vi "SID_adsr.vi"(0 "status in":T3(ring), 1 "Reg":T2, 5 "acc in":T1) -> (4 "status out":T3(ring), 6 "acc out":T1)   [LabVIEW 2018]
uses:
  SID_voice_reg.ctl
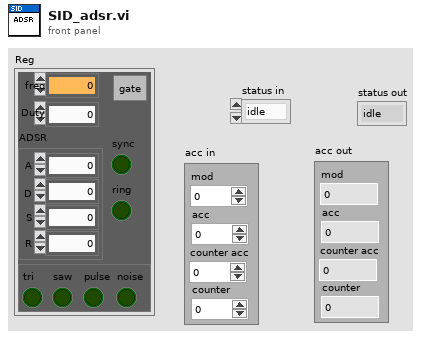
[diagram p1: front panel]
types:
  T1 = cluster{"mod":dbl, "acc":dbl, "counter acc":dbl, "counter":i32}
  T2 = typedef "SID_voice_reg.ctl" = cluster{"freq":dbl, "gate":bool, "ADSR":cluster{"A":dbl, "D":dbl, "S":dbl, "R":dbl}, "Duty":dbl, "osc enab":cluster{"tri":bool, "saw":bool, "pulse":bool, "noise":bool}, "sync":bool, "ring":bool}
  T3 = enum16{"idle", "pre-attack", "attack", "pre-decay", "decay", "sustain", "pre-release", "release"}
  T4 = cluster{"mod in":dbl, "acc in":dbl, "counter acc in":dbl, "counter in":i32}
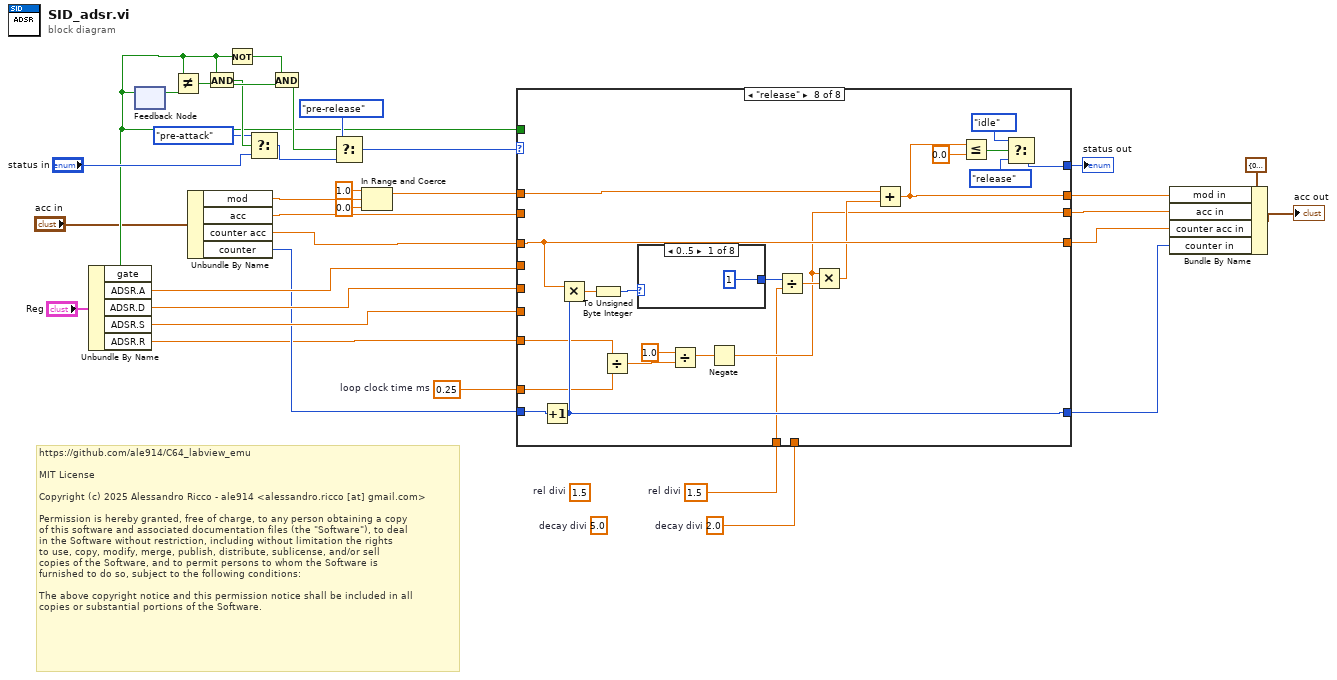
[diagram p0: block diagram]
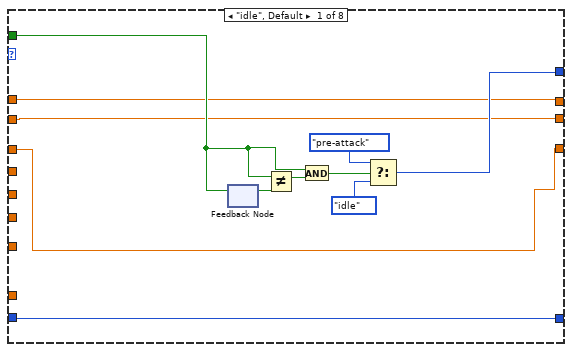
[diagram p2: hidden frame]
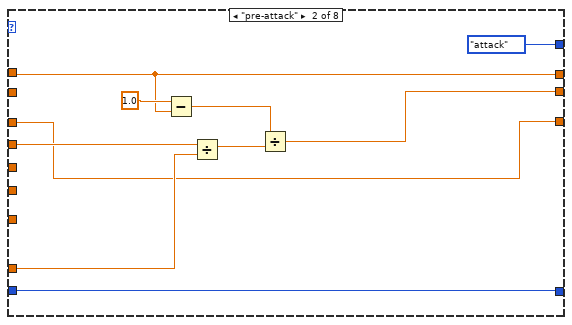
[diagram p3: hidden frame]
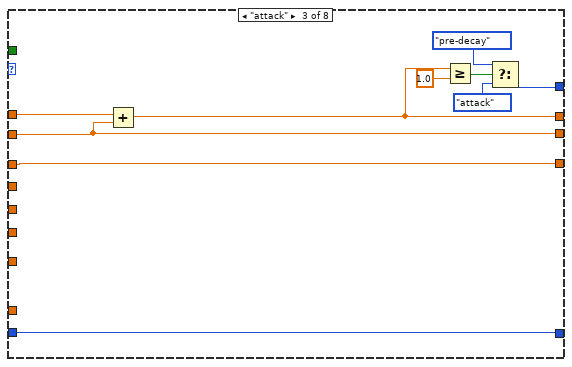
[diagram p4: hidden frame]
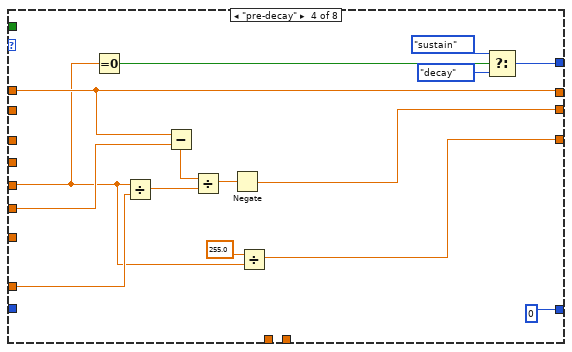
[diagram p5: hidden frame]
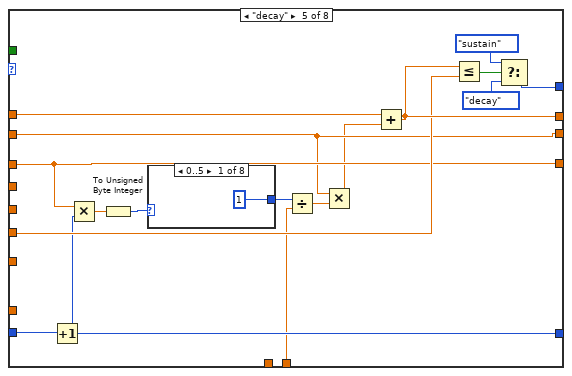
[diagram p6: hidden frame]
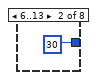
[diagram p7: hidden frame]
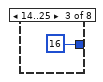
[diagram p8: hidden frame]
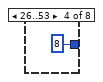
[diagram p9: hidden frame]
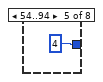
[diagram p10: hidden frame]
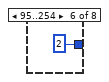
[diagram p11: hidden frame]
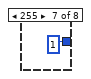
[diagram p12: hidden frame]
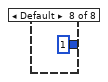
[diagram p13: hidden frame]
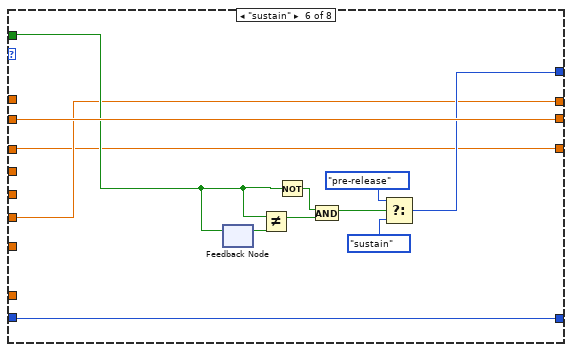
[diagram p14: hidden frame]
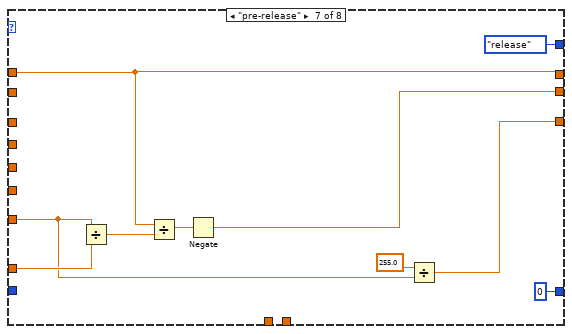
[diagram p15: hidden frame]
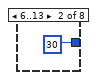
[diagram p16: hidden frame]
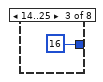
[diagram p17: hidden frame]
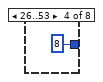
[diagram p18: hidden frame]
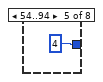
[diagram p19: hidden frame]
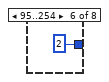
[diagram p20: hidden frame]
diagram:
  (unwired) 5.0  # decay divi
  (unwired) 1.5  # rel divi
  w1 = 2.0  # decay divi
  w2 = 1.5  # rel divi
  w22 = 0.25  # loop clock time ms
  # "https://github.com/ale914/C64_labview_emu\n\nMIT License\n\nCopyright (c) 2025 Alessandro Ricco - ale914 <alessandro.ricco [at] gmail.com>\n\nPermission is hereby granted, free of charge, to any person obtaining a copy\nof this software and associated documentation files (the \"Software\"), to deal\nin the Software without restriction, including without limitation the rights\nto use, copy, modify, merge, publish, distribute, sublicense, and/or sell\ncopies of the Software, and to permit persons to whom the Software is\nfurnished to do so, subject to the following conditions:\n\nThe above copyright notice and this permission notice shall be included in all\ncopies or substantial portions of the Software."
  n1 = Unbundle By Name("Reg") -> ("gate"=w17:bool, "ADSR.A"=w20:dbl, "ADSR.D"=w19:dbl, "ADSR.S"=w18:dbl, "ADSR.R"=w4:dbl)
  n2 = feedback #1() -> (w33:bool)  [unwired: 1 in]
  n3 = feedback-in #1(w17) -> ()
  n4 = Not Equal?(x=w17, y=w33) -> (x != y?=w32:bool)
  n5 = Unbundle By Name("acc in") -> ("mod"=w14:dbl, "acc"=w13:dbl, "counter acc"=w12:dbl, "counter"=w11:i32)
  n6 = And(x=w17, y=w32) -> (x .and. y?=w30:bool)
  n7 = Not(x=w17) -> (.not. x?=w31:bool)
  n8 = Select(t=T3."pre-attack", s=w30, f="status in") -> (s? t:f=w27:T3)
  n9 = And(x=w31, y=w32) -> (x .and. y?=w23:bool)
  n10 = Select(t=T3."pre-release", s=w23, f=w27) -> (s? t:f=w16:T3)
  n11 = In Range and Coerce(upper limit=1.0, x=w14, lower limit=0.0) -> (coerced(x)=w24:dbl)  [unwired: 1 out]
  n12 = case shown="\"release\"" w16 {
    tunnel: [w37 w55 w64 w79 w83 w117 w124 w129] -> w9
    tunnel: w13 -> [w37 _ w64 _ w83 w117 _ _]
    tunnel: w24 -> [w38 w49 w65 w73 w97 _ w118 w145]
    tunnel: [w38 w49 w63 w73 w92 w108 w118 w143] -> w10
    tunnel: [w40 T3."attack" w58 w77 w93 w109 T3."release" w144] -> w34
    tunnel: w17 -> [w39 _ _ _ _ w114 _ _]
    tunnel: w20 -> [_ w52 _ _ _ _ _ _]
    tunnel: w19 -> [_ _ _ w66 _ _ _ _]
    tunnel: w18 -> [_ _ _ w72 w91 w108 _ _]
    tunnel: w4 -> [_ _ _ _ _ _ w121 w132]
    tunnel: w22 -> [_ w51 _ w74 _ _ w123 w131]
    tunnel: [w36 w47 w57 w70 w88 w106 w120 w137] -> w8
    tunnel: w12 -> [w36 w47 w57 _ w88 w106 _ w137]
    tunnel: w11 -> [w35 w46 w56 _ w87 w107 _ w138]
    tunnel: [w35 w46 w56 0 w86 w107 0 ("counter in") w136] -> w7
    tunnel: w2 -> [_ _ _ _ _ _ _ w128]
    tunnel: w1 -> [_ _ _ _ w81 _ _ _]
    frame "idle", Default {
      n13 = feedback #2() -> (w45:bool)  [unwired: 1 in]
      n14 = feedback-in #2(w39) -> ()
      n15 = Not Equal?(x=w39, y=w45) -> (x != y?=w44:bool)
      n16 = And(x=w39, y=w44) -> (x .and. y?=w43:bool)
      n17 = Select(t=T3."pre-attack", s=w43, f=T3."idle") -> (s? t:f=w40:T3)
    }
    frame "pre-attack" {
      n18 = Subtract(x=1.0 ("y"), y=w49) -> (x-y=w48:dbl)
      n19 = Divide(x=w52, y=w51) -> (x/y=w54:dbl)
      n20 = Divide(x=w48, y=w54) -> (x/y=w55:dbl)
    }
    frame "attack" {
      n21 = Add(x=w65, y=w64) -> (x+y=w63:dbl)
      n22 = Greater Or Equal?(x=w63, y=1.0) -> (x >= y?=w59:bool)
      n23 = Select(t=T3."pre-decay", s=w59, f=T3."attack") -> (s? t:f=w58:T3)
    }
    frame "pre-decay" {
      n24 = Equal To 0?(x=w66) -> (x = 0?=w76:bool)
      n25 = Divide(x=w66, y=w74) -> (x/y=w80:dbl)
      n26 = Subtract(x=w73, y=w72) -> (x-y=w68:dbl)
      n27 = Divide(x=w68, y=w80) -> (x/y=w67:dbl)
      n28 = Negate(x=w67) -> (-x=w79:dbl)
      n29 = Divide(x=255.0 ("y"), y=w66) -> (x/y=w70:dbl)
      n30 = Select(t=T3."sustain", s=w76, f=T3."decay") -> (s? t:f=w77:T3)
    }
    frame "decay" {
      n31 = Increment(x=w87) -> (x+1=w86:i32)
      n32 = Multiply(x=w88, y=w86) -> (x*y=w85:dbl)
      n33 = To Unsigned Byte Integer(number=w85) -> (unsigned 8bit integer=w90:u8)
      n34 = case shown="0..5" w90 {
        tunnel: [u8 1 ("exp_period") u8 30 ("exp_period") u8 16 ("exp_period") u8 8 ("exp_period") u8 4 ("exp_period") u8 2 ("exp_period") u8 1 ("exp_period") u8 1 ("exp_period")] -> w89
        frame 0..5 {
          (unwired) TRUE ("hold zero")
        }
        frame 6..13 {
        }
        frame 14..25 {
        }
        frame 26..53 {
        }
        frame 54..94 {
        }
        frame 95..254 {
        }
        frame 255 {
        }
        frame Default {
        }
      }
      n35 = Divide(x=w89, y=w81) -> (x/y=w84:dbl)
      n36 = Multiply(x=w83, y=w84) -> (x*y=w82:dbl)
      n37 = Add(x=w97, y=w82) -> (x+y=w92:dbl)
      n38 = Less Or Equal?(x=w92, y=w91) -> (x <= y?=w94:bool)
      n39 = Select(t=T3."sustain", s=w94, f=T3."decay") -> (s? t:f=w93:T3)
    }
    frame "sustain" {
      n40 = feedback #3() -> (w116:bool)  [unwired: 1 in]
      n41 = feedback-in #3(w114) -> ()
      n42 = Not Equal?(x=w114, y=w116) -> (x != y?=w115:bool)
      n43 = Not(x=w114) -> (.not. x?=w113:bool)
      n44 = And(x=w113, y=w115) -> (x .and. y?=w110:bool)
      n45 = Select(t=T3."pre-release", s=w110, f=T3."sustain") -> (s? t:f=w109:T3)
    }
    frame "pre-release" {
      n46 = Divide(x=w121, y=w123) -> (x/y=w126:dbl)
      n47 = Divide(x=w118, y=w126) -> (x/y=w125:dbl)
      n48 = Negate(x=w125) -> (-x=w124:dbl)
      n49 = Divide(x=255.0 ("y"), y=w121) -> (x/y=w120:dbl)
    }
    frame "release" {
      n50 = Increment(x=w138) -> (x+1=w136:i32)
      n51 = Multiply(x=w137, y=w136) -> (x*y=w140:dbl)
      n52 = To Unsigned Byte Integer(number=w140) -> (unsigned 8bit integer=w142:u8)
      n53 = Divide(x=w132, y=w131) -> (x/y=w134:dbl)
      n54 = case shown="0..5" w142 {
        tunnel: [u8 1 ("exp_period") u8 30 ("exp_period") u8 16 ("exp_period") u8 8 ("exp_period") u8 4 ("exp_period") u8 2 ("exp_period") u8 1 ("exp_period") u8 1 ("exp_period")] -> w141
        frame 0..5 {
          (unwired) TRUE ("hold zero")
        }
        frame 6..13 {
        }
        frame 14..25 {
        }
        frame 26..53 {
        }
        frame 54..94 {
        }
        frame 95..254 {
        }
        frame 255 {
        }
        frame Default {
        }
      }
      n55 = Divide(x=1.0, y=w134) -> (x/y=w133:dbl)
      n56 = Negate(x=w133) -> (-x=w129:dbl)
      n57 = Divide(x=w141, y=w128) -> (x/y=w139:dbl)
      n58 = Multiply(x=w129, y=w139) -> (x*y=w135:dbl)
      n59 = Add(x=w145, y=w135) -> (x+y=w143:dbl)
      n60 = Less Or Equal?(x=w143, y=0.0) -> (x <= y?=w148:bool)
      n61 = Select(t=T3."idle", s=w148, f=T3."release") -> (s? t:f=w144:T3)
    }
  }
  "status out" <- w34
  n62 = Bundle By Name(cluster=T4 {"mod in"=0.0, "acc in"=0.0, "counter acc in"=0.0, "counter in"=0} ("acc out"), "mod in"=w10, "acc in"=w9, "counter acc in"=w8, "counter in"=w7) -> (→"acc out":T4)
